vi "DAC Configure.vi"(8 "error in":errorcluster, 11 "DAC ADV in":refnum<class "DAC ADV.lvclass">) -> (0 "error out":errorcluster, 3 "DAC ADV out":refnum<class "DAC ADV.lvclass">)   [LabVIEW 2019, in "DAC.lvlib" / "DAC ADV.lvclass"]
uses:
  DAC ADV.lvclass
  C:/Users/wg/Documents/LV_Projects/test-stand/App/DAC/DAC.lvclass
  DAC.lvclass/DAC.ctl
  DAC ADV.lvclass/DAC ADV.ctl
  DAC.lvclass
  <vilib>/Instr/_visa.llb/VISA Configure Serial Port (Instr).vi
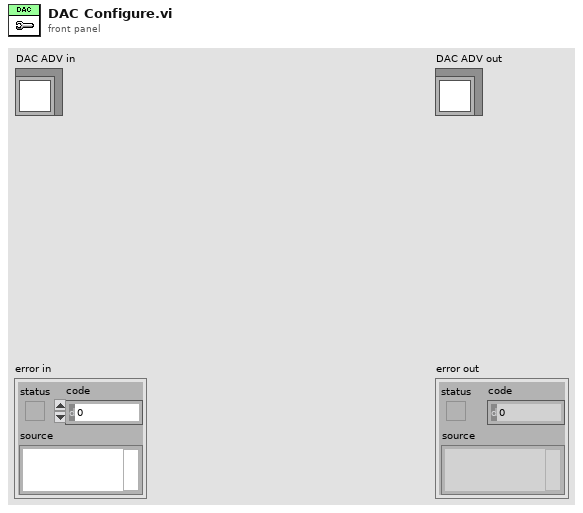
[diagram p1: front panel]
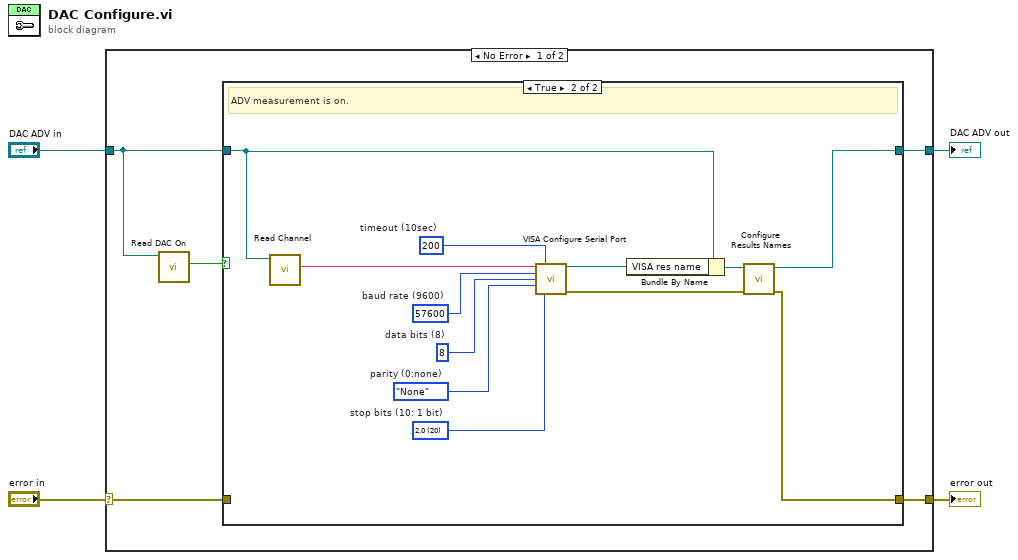
[diagram p0: block diagram]
diagram:
  n1 = case shown="No Error" "error in" {
    selector: "error in" -> [w6 w25]
    tunnel: [w5 w25] -> w4
    tunnel: [w7 w24] -> w3
    tunnel: "DAC ADV in" -> [w9 w24]
    frame No Error {
      n2 = call "Read DAC On.vi"("DAC in"=w9) -> ("DAC On"=w8:bool)  [unwired: 8 in, 2 out]
      n3 = case shown="True" w8 {
        tunnel: w9 -> [w11 w19]
        tunnel: [w11 w23] -> w7
        tunnel: w6 -> [w10 _]
        tunnel: [w10 w20] -> w5
        frame False {
          # "ADV measurement is off."
        }
        frame True {
          w13 = u32 200  # timeout (10sec)
          w14 = u16 20 items=["1.0"=10, "1.5"=15, "2.0"=20]  # stop bits (10: 1 bit)
          w15 = enum16{"None", "Odd", "Even", "Mark", "Space"}."None"  # parity (0:none)
          w16 = u16 8  # data bits (8)
          w17 = u32 57600  # baud rate (9600)
          # "ADV measurement is on."
          n4 = call "Read Channel.vi"("DAC in"=w19) -> ("Channel"=w18:string)  [unwired: 8 in, 2 out]
          n5 = call-poly "VISA Configure Serial Port"("VISA resource name"=w18, "timeout (10sec)"=w13, "baud rate (9600)"=w17, "data bits (8)"=w16, "parity (0:none)"=w15, "stop bits (10: 1 bit)"=w14) -> ("VISA resource name out"=w12:refnum<visa-resource-name>, "error out"=w21:errorcluster)  [unwired: 8 in]
          n6 = Bundle By Name(cluster=w19, "VISA res name"=w12) -> (w22:refnum<class "DAC ADV.lvclass">)
          n7 = call "Configure Results Names.vi"("error in"=w21, "DAC ADV in"=w22) -> ("error out"=w20:errorcluster, "DAC ADV out"=w23:refnum<class "DAC ADV.lvclass">)  [unwired: 8 in]
        }
      }
    }
    frame Error {
    }
  }
  "error out" <- w4
  "DAC ADV out" <- w3
